vi "SC Get Tool Values.vi"(9 "tool lines":string[](array[string]), 10 "key":string) -> (1 "values":string[](array[string]))   [LabVIEW 2023]
doc: "Returns the rest of every SYSTEMCORE-TOOL line that starts with key (e.g. LOCAL_ONLY), in order."
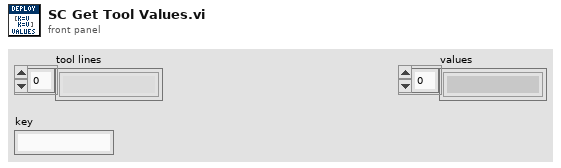
[diagram p1: front panel]
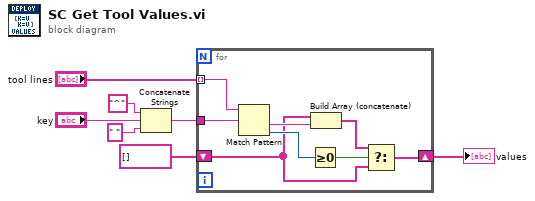
[diagram p0: block diagram]
diagram:
  n1 = Concatenate Strings("^", "key", " ") -> (w3:string)
  n2 = for {
    tunnel: "tool lines" -> [w15] mode=indexing
    tunnel: w3 -> [w14]
    shift-right: [w8] -> w2
    shift-left: string[] [] -> [w9]
    n3 = Match Pattern(string=w15, regular expression=w14) -> (after substring=w12:string, offset past match=w13:i32)  [unwired: 1 in, 2 out]
    n4 = Greater Or Equal To 0?(x=w13) -> (x >= 0?=w11:bool)
    n5 = Build Array (concatenate)(w9, w12) -> (w10:string[])
    n6 = Select(t=w10, s=w11, f=w9) -> (s? t:f=w8:string[])
  }
  "values" <- w2
